vi "VIEW.vi"() -> ()   [LabVIEW 2013, in "VIEW.lvclass"]
uses:
  VIEW.lvclass
  Controller/base/CONTROLLER.lvclass
panel:
  out "error out":errorcluster
  in  "stop":bool
  in  "ctrl2":string
  in  "DoAction1":bool
  in  "Enqueue Element":bool
  in  "mystring":string
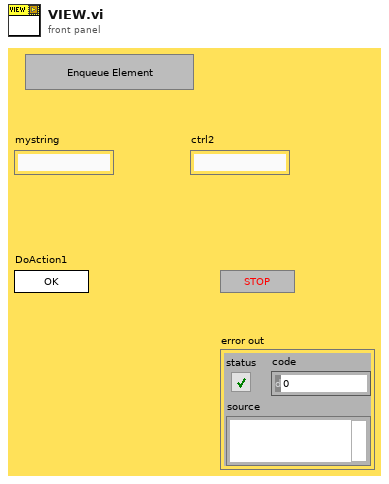
[diagram p1: front panel]
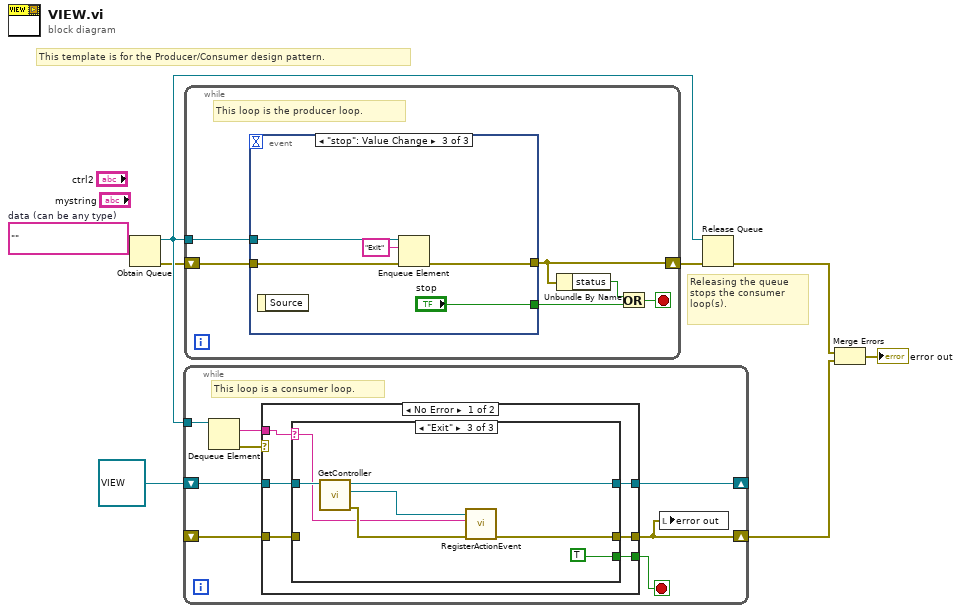
[diagram p0: block diagram]
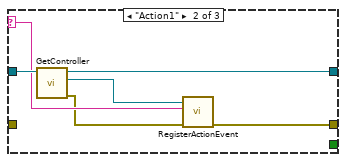
[diagram p3: hidden frame]
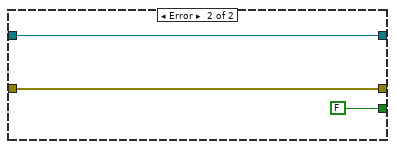
[diagram p4: hidden frame]
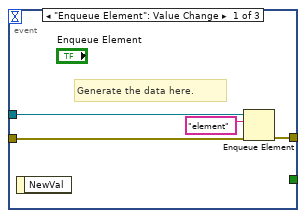
[diagram p5: hidden frame]
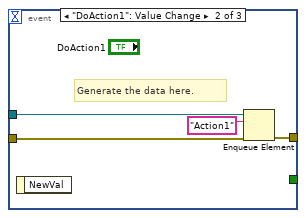
[diagram p6: hidden frame]
diagram:
  w6 = ""  # data (can be any type)
  # "Releasing the queue stops the consumer loop(s)."
  # "This template is for the Producer/Consumer design pattern."
  n1 = Obtain Queue(element data type=w6) -> (queue out=w7:refnum<queue>, error out=w4:errorcluster)  [unwired: 4 in, 1 out]
  n2 = while {
    tunnel: w7 -> [w16]
    shift-right: [w11] -> _
    shift-left: refnum<class "VIEW.lvclass"> refnum ("VIEW.lvclass") -> [w12]
    shift-right: [w9] -> w1
    shift-left: _ -> [w10]
    stop <- w13 stop-if-true
    # "This loop is a consumer loop."
    n3 = Dequeue Element(queue=w16) -> (element=w14:string, error out=w15:errorcluster)  [unwired: 2 in, 2 out]
    n4 = case shown="No Error" w15 {
      tunnel: w14 -> [w22 _]
      tunnel: [w19 FALSE] -> w13
      tunnel: w12 -> [w21 w39]
      tunnel: [w20 w39] -> w11
      tunnel: [w18 w38] -> w9
      tunnel: w10 -> [w17 w38]
      frame No Error {
        n5 = case shown="\"Exit\"" w22 {
          selector: w22 -> [_ w27 w32]
          tunnel: w21 -> [w24 w30 w37]
          tunnel: [w24 w28 w35] -> w20
          tunnel: [_ _ TRUE] -> w19
          tunnel: [w23 w25 w31] -> w18
          tunnel: w17 -> [w23 _ _]
          frame "False", Default {
          }
          frame "Action1" {
            n6 = call-dynamic "GetController.vi"("VIEW in"=w30) -> ("error out"=w26:errorcluster, "CONTROLLER"=w29:refnum<class "CONTROLLER.lvclass">, "VIEW out"=w28:refnum<class "VIEW.lvclass">)  [unwired: 8 in]
            n7 = call "RegisterActionEvent.vi"("error in (no error)"=w26, "Action"=w27, "CONTROLLER in"=w29) -> ("error out"=w25:errorcluster)  [unwired: 7 in, 1 out]
          }
          frame "Exit" {
            n8 = call-dynamic "GetController.vi"("VIEW in"=w37) -> ("error out"=w33:errorcluster, "CONTROLLER"=w36:refnum<class "CONTROLLER.lvclass">, "VIEW out"=w35:refnum<class "VIEW.lvclass">)  [unwired: 8 in]
            n9 = call "RegisterActionEvent.vi"("error in (no error)"=w33, "Action"=w32, "CONTROLLER in"=w36) -> ("error out"=w31:errorcluster)  [unwired: 7 in, 1 out]
          }
        }
      }
      frame Error {
      }
    }
    n10 = local write "error out"(w9) -> ()
  }
  n11 = while {
    shift-right: [w42] -> w5
    shift-left: w4 -> [w45]
    tunnel: w7 -> [w46]
    stop <- w43 stop-if-true
    # "This loop is the producer loop."
    n12 = event shown="[2] \"stop\": Value Change" {
      selector: _ -> [_ _ _]
      dyn-events: _ -> [_ _ _]
      timeout: _ -> [_ _ _]
      tunnel: w46 -> [w50 w54 w56]
      tunnel: w45 -> [w49 w53 w58]
      tunnel: [w48 w52 w57] -> w42
      tunnel: [_ _ "stop"] -> w44
      event "Enqueue Element": Value Change {
        # "Generate the data here."
        n13 = event-data() -> ()  [unwired: 1 in, 1 out]
        n14 = Enqueue Element(queue=w50, element="element", error in (no error)=w49) -> (error out=w48:errorcluster)  [unwired: 1 in, 2 out]
      }
      event "DoAction1": Value Change {
        # "Generate the data here."
        n15 = event-data() -> ()  [unwired: 1 in, 1 out]
        n16 = Enqueue Element(queue=w54, element="Action1", error in (no error)=w53) -> (error out=w52:errorcluster)  [unwired: 1 in, 2 out]
      }
      event "stop": Value Change {
        n17 = event-data() -> ()  [unwired: 1 in, 1 out]
        n18 = Enqueue Element(queue=w56, element="Exit", error in (no error)=w58) -> (error out=w57:errorcluster)  [unwired: 1 in, 2 out]
      }
    }
    n19 = Unbundle By Name(w42) -> ("status"=w41:bool)
    n20 = Or(x=w41, y=w44) -> (x .or. y?=w43:bool)
  }
  n21 = Release Queue(queue=w7, error in (no error)=w5) -> (error out=w2:errorcluster)  [unwired: 1 in, 2 out]
  n22 = Merge Errors(w2, w1) -> (→"error out":errorcluster)
